vi "check IDN Query Value.vi"(8 "error in (no error)":errorcluster, 11 "NR in":refnum<class "NR.lvclass">) -> (0 "error out":errorcluster, 2 "Connected":bool, 3 "NR out":refnum<class "NR.lvclass">)   [LabVIEW 2023, in "ANRITSU Call Box.lvlib" / "NR.lvclass"]
uses:
  NR.lvclass
  NR.lvclass/NR.ctl
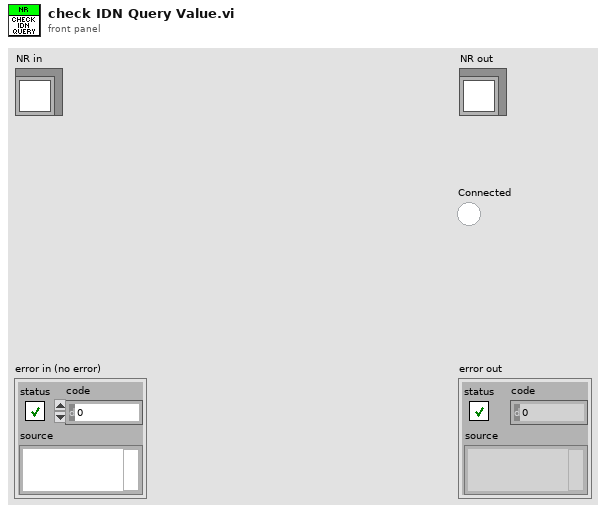
[diagram p1: front panel]
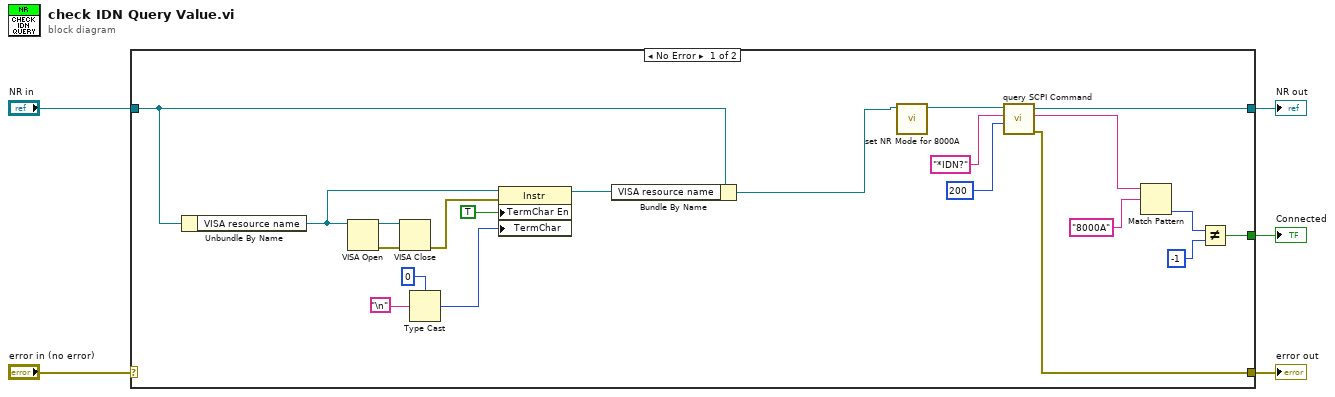
[diagram p0: block diagram]
diagram:
  n1 = case shown="No Error" "error in (no error)" {
    selector: "error in (no error)" -> [_ w28]
    tunnel: [w11 w28] -> w4
    tunnel: [w9 w27] -> w2
    tunnel: "NR in" -> [w19 w27]
    tunnel: [w10 _] -> w1
    frame No Error {
      n2 = Unbundle By Name(w19) -> ("VISA resource name"=w25:refnum<visa-resource-name>)
      n3 = VISA Open(VISA resource name=w25) -> (VISA resource name=w8:refnum<visa-resource-name>, error out=w26:errorcluster)  [unwired: 4 in]
      n4 = VISA Close(VISA resource name=w8, error in (no error)=w26) -> (error out=w24:errorcluster)
      n5 = Type Cast(type=u8 0 ("Message Based Settings:Termination Character"), x="\n") -> (*(type *) &x=w20:u8)
      n6 = property class="Instr"(reference=w25, error in=w24, "TermChar En"=TRUE ("Message Based Settings:Termination Character Enable"), "TermChar"=w20) -> (reference out=w18:refnum<visa-resource-name>)  [unwired: 1 out]
      n7 = Bundle By Name(cluster=w19, "VISA resource name"=w18) -> (w7:refnum<class "NR.lvclass">)
      n8 = call "set NR Mode for 8000A.vi"("NR in"=w7) -> ("NR out"=w6:refnum<class "NR.lvclass">)  [unwired: 9 in, 1 out]
      n9 = call "query SCPI Command.vi"("Read Buffer Length"=u32 200, "SCPI Command"="*IDN?" ("write buffer"), "NR in"=w6) -> ("error out"=w11:errorcluster, "Read Buffer String"=w15:string, "NR out"=w9:refnum<class "NR.lvclass">)  [unwired: 6 in]
      n10 = Match Pattern(string=w15, regular expression="8000A") -> (offset past match=w13:i32)  [unwired: 1 in, 3 out]
      n11 = Not Equal?(x=w13, y=-1) -> (x != y?=w10:bool)
    }
    frame Error {
    }
  }
  "error out" <- w4
  "NR out" <- w2
  "Connected" <- w1
